vi "ASD Baseline substract VI.vi"(8 "Baseline":dbl[](array[numeric]), 11 "Region Raw":dbl[](array[numeric])) -> (3 "Substracted Raw data":dbl[](array[numeric]))   [LabVIEW 2018]
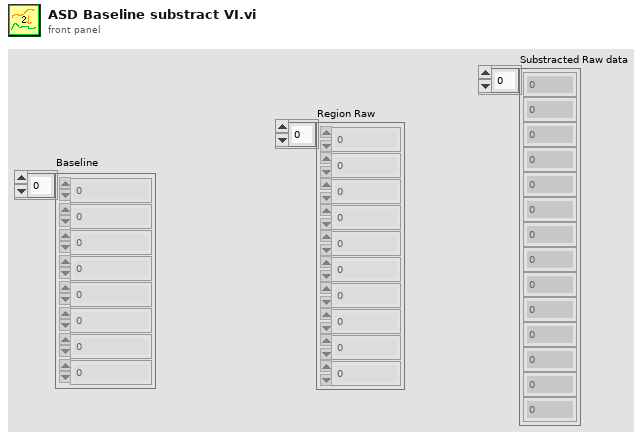
[diagram p1: front panel]
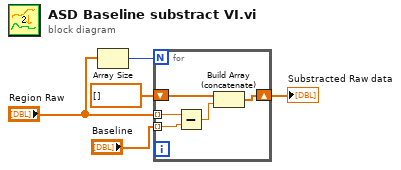
[diagram p0: block diagram]
diagram:
  n1 = Array Size(array="Region Raw") -> (size(s)=w5:i32)
  n2 = for {
    N: w5 -> [_]
    tunnel: "Baseline" -> [w9] mode=indexing
    tunnel: "Region Raw" -> [w10] mode=indexing
    shift-right: [w7] -> w1
    shift-left: dbl[] [] -> [w6]
    n3 = Subtract(x=w10, y=w9) -> (x-y=w8:dbl)
    n4 = Build Array (concatenate)(w6, w8) -> (w7:dbl[])
  }
  "Substracted Raw data" <- w1
